vi "Test_pgJDP_built.vi"() -> ()   [LabVIEW 2020]
uses:
  <vilib>/Viviota/shared/ORM.lvlibp/TypeMap/TypeMap.lvclass
  <vilib>/Viviota/shared/ORM_pgsql_jdp.lvlibp/dbc/DBC.lvclass
  C:/Program Files/National Instruments/LabVIEW 2020/vi.lib/Viviota/shared/ORM.lvlibp/DbConnection/DbConnection.lvclass
  <vilib>/Viviota/shared/ORM_pgsql_jdp.lvlibp/PGJDPMapper/PGJDPMapper.lvclass
  C:/Program Files/National Instruments/LabVIEW 2020/vi.lib/Viviota/shared/ORM.lvlibp/SqlMapper/SqlMapper.lvclass
  <vilib>/Viviota/shared/ORM_lib.lvlibp/ObjectRow/ObjectLUT.lvclass
  <vilib>/numeric/Random Number (Range) I64.vi
  <vilib>/numeric/Random Number (Range) DBL.vi
  f3693442-7653-4e44-a421-498bef5f0c13.vi
  <vilib>/Analysis/baseanly.llb/Mean (DBL).vi
  <vilib>/numeric/sub_Random U32.vi
  <vilib>/JDP Science/JSONtext/Variant to JSON Text.vi
  <vilib>/Viviota/shared/ORM_lib.lvlibp/ObjectRow/Write LUT.vi
  <vilib>/Viviota/shared/ORM.lvlibp/DbConnection/Write SupportTX.vi
  <vilib>/Viviota/shared/ORM.lvlibp/SqlMapper/Write DbConnection.vi
  <vilib>/Viviota/shared/ORM.lvlibp/TypeMap/Write Table Name.vi
  <vilib>/Viviota/shared/ORM.lvlibp/TypeMap/Write Autokey.vi
  <vilib>/Viviota/shared/ORM_lib.lvlibp/ObjectRow/Read LUT.vi
  <vilib>/JDP Science/JSONtext/LVClass Serializer/JSONtext LVClass Serializer.lvclass
  <vilib>/Analysis/NI_AALBase.lvlib
panel:
  out "mean 3":dbl format="%0.6f"
  out "mean 2":dbl format="%0.6f"
  out "mean":dbl format="%0.6f"
  out "x-y":dbl[](array[numeric])
  out "Array 2":dbl[](array[numeric])
  out "Array":dbl[](array[numeric])
  out "LUT 2":variant[](array[variant])
  out "LUT":variant[](array[variant])
  out "id":i32[](array[numeric])
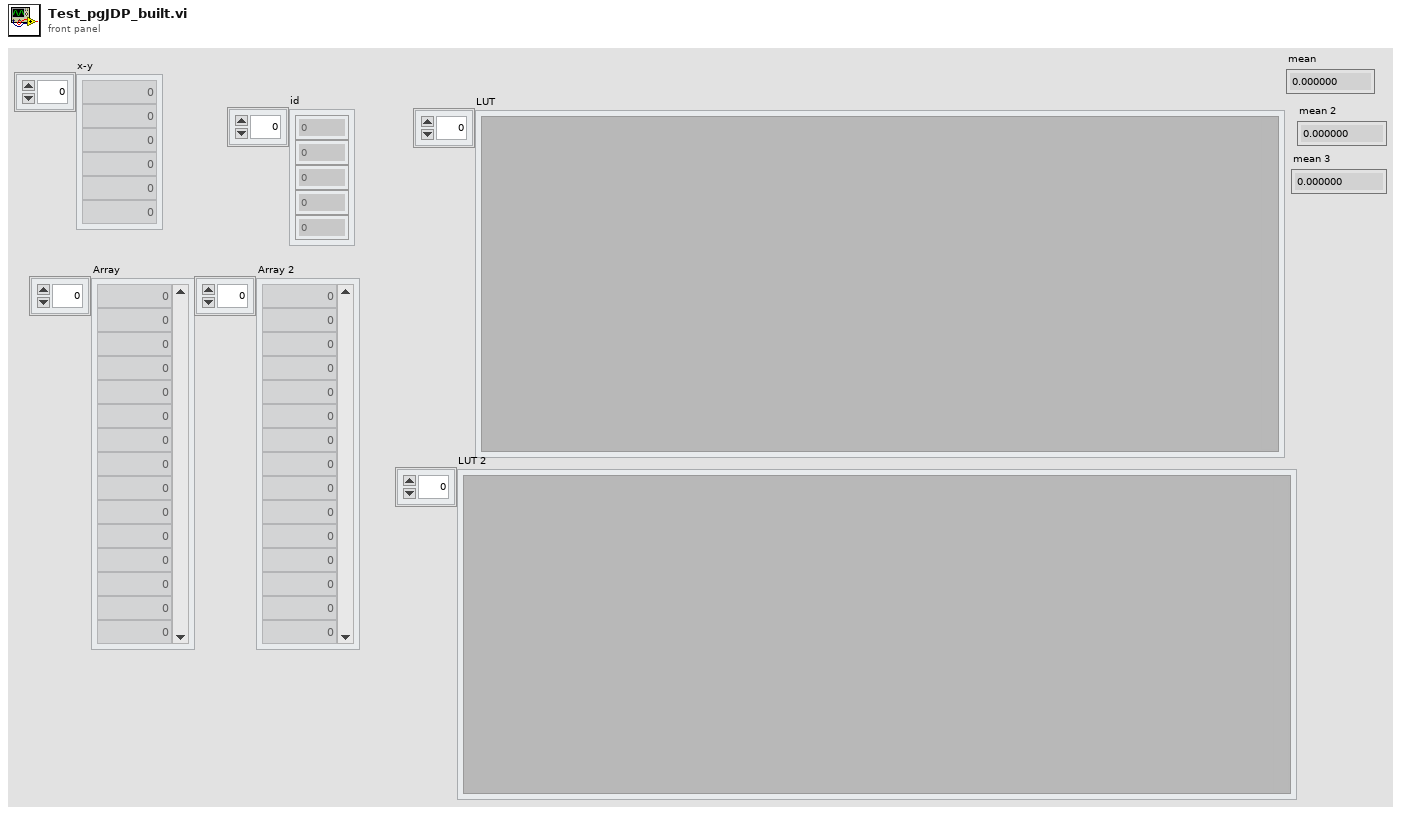
[diagram p1: front panel]
types:
  T1 = cluster{"Text":string, "Integer":i32, "dbl":dbl, "timestamp":timestamp}
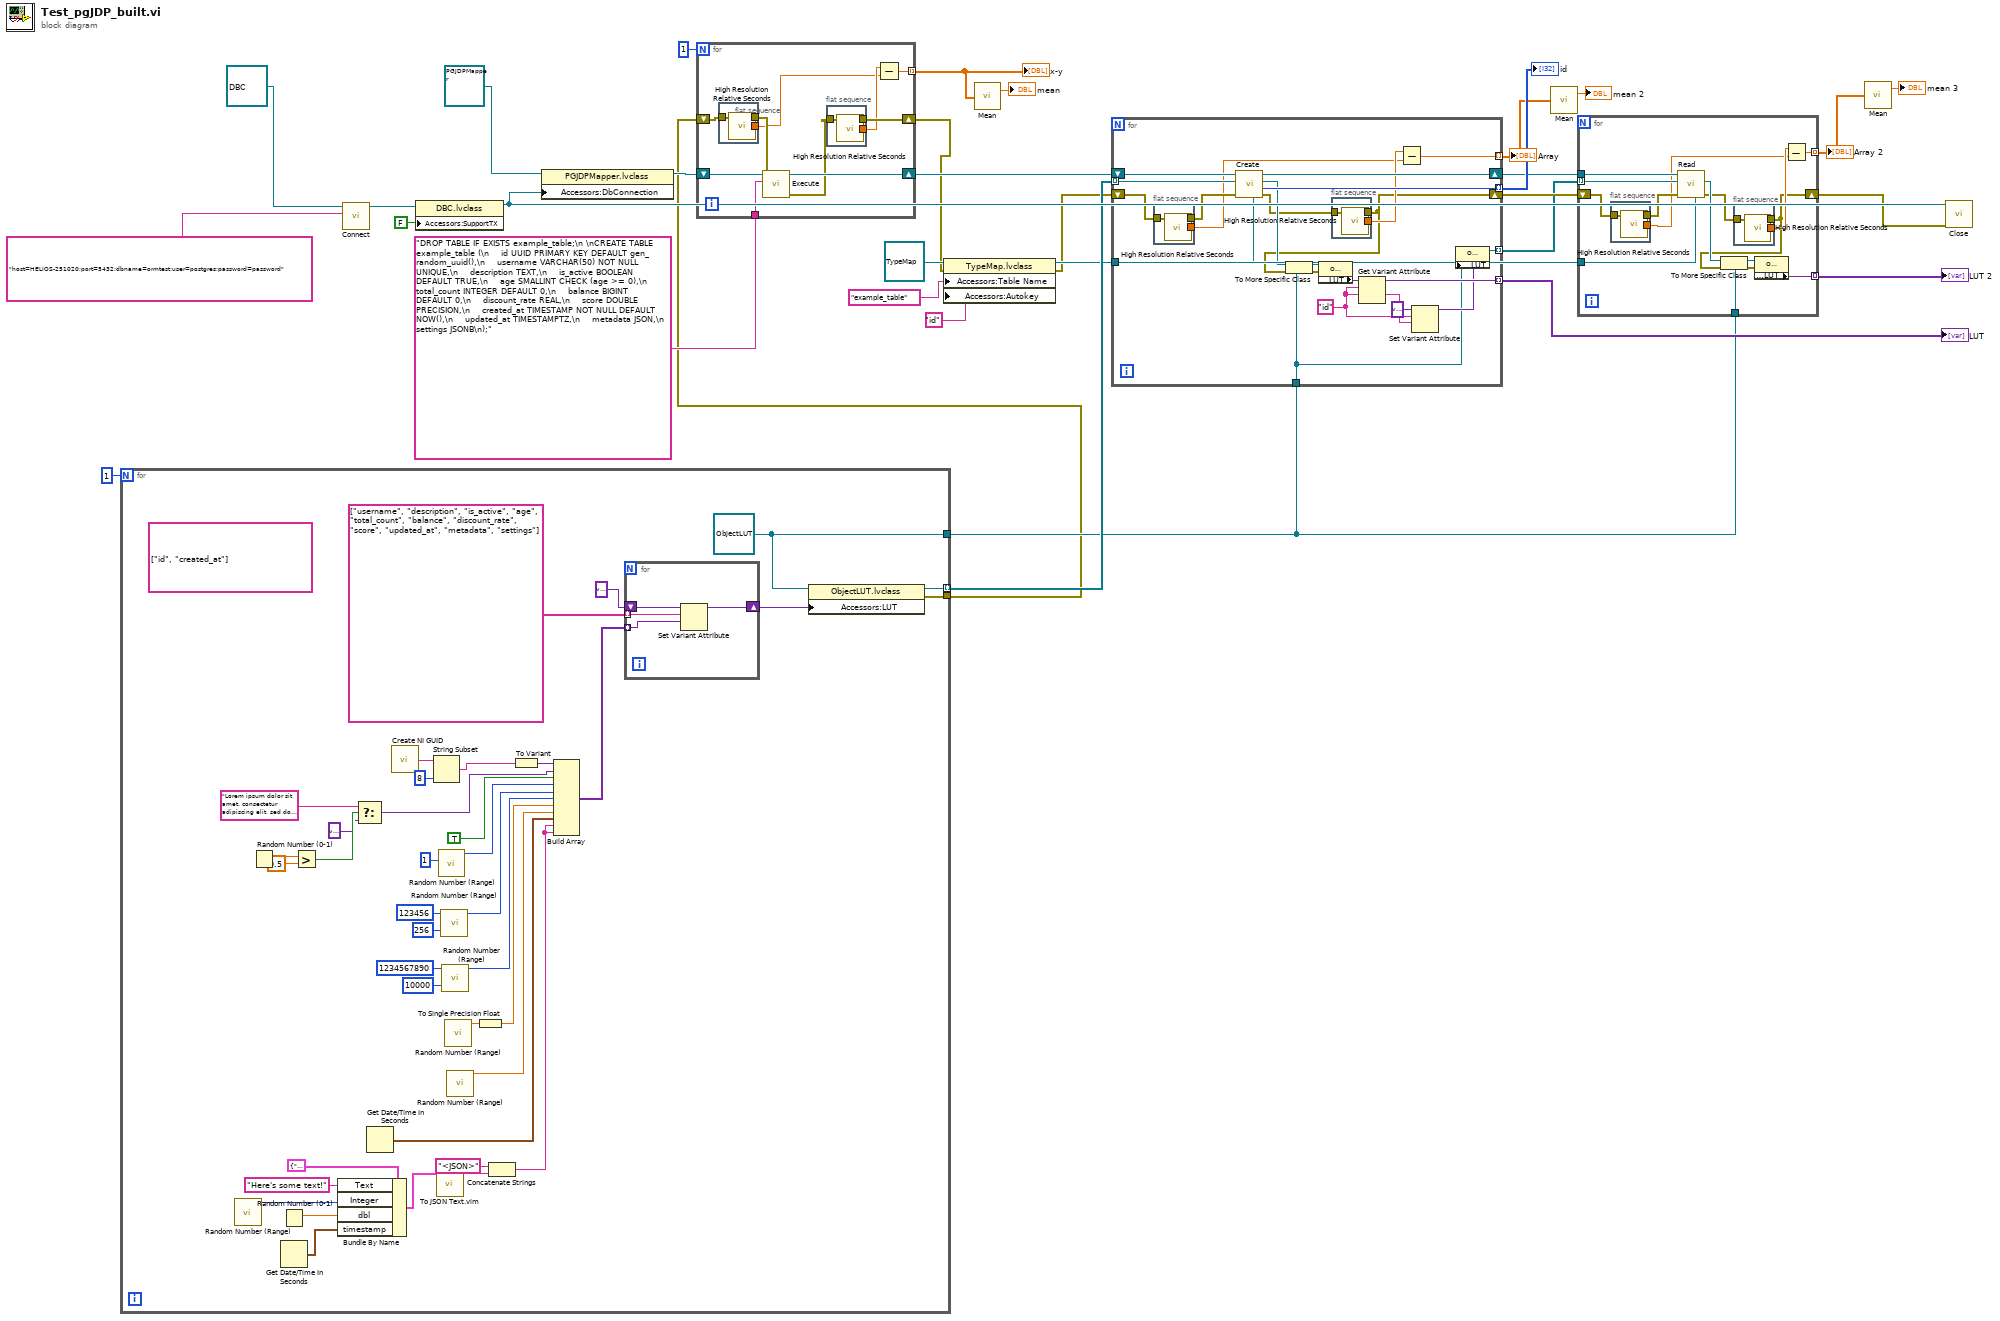
[diagram p0: block diagram]
diagram:
  n1 = for {
    N: 1 -> [_]
    tunnel: [w42] -> w27 mode=indexing
    tunnel: [w41] -> w17
    tunnel: [w36] -> w12
    w41 = refnum<class "ObjectLUT.lvclass"> refnum ("ORM_lib.lvlibp:ObjectLUT.lvclass")
    (unwired) string[] ["id", "created_at"]
    n2 = call-poly <vilib>:"Random Number (Range).vi"() -> ("number"=w49:i64)  [unwired: 11 in]
    n3 = Random Number (0-1)() -> (number: 0 to 1=w57:dbl)
    n4 = Random Number (0-1)() -> (number: 0 to 1=w50:dbl)
    n5 = Get Date/Time In Seconds() -> (seconds since 1Jan1904=w51:timestamp)
    n6 = Greater?(x=w57, y=0.5) -> (0:w55:bool)
    n7 = Bundle By Name(cluster=T1 {"Text"="This is a test", "Integer"=0, "dbl"=0.0, "timestamp"=timestamp(0 s since 1904-01-01)}, "Text"="Here's some text!", "Integer"=w49, "dbl"=w50, "timestamp"=w51) -> (w47:T1)
    n8 = Select(t="Lorem ipsum dolor sit amet, consectetur adipiscing elit, sed do eiusmod tempor incididunt ut labore et dolore magna aliqua", s=w55, f=variant) -> (s? t:f=w34:variant)
    n9 = Get Date/Time In Seconds() -> (seconds since 1Jan1904=w48:timestamp)
    n10 = call <vilib>:"Create NI GUID.vi"() -> ("NI GUID"=w72:string)
    n11 = String Subset(string=w72, length (rest)=8 ("length (rest)")) -> (substring=w67:string)  [unwired: 1 in]
    n12 = call "To JSON Text.vim"("Anything"=w47) -> ("<JSON>"=w40:string)  [unwired: 9 in, 1 out]
    n13 = call-poly <vilib>:"Random Number (Range).vi"("lower bound (-100)"=i64 1) -> ("number"=w64:i64)  [unwired: 10 in]
    n14 = call-poly <vilib>:"Random Number (Range).vi"("lower bound (-100)"=i64 256, "upper bound (100)"=i64 123456) -> ("number"=w63:i64)  [unwired: 9 in]
    n15 = call-poly <vilib>:"Random Number (Range).vi"("lower bound (-100)"=i64 10000, "upper bound (100)"=i64 1234567890) -> ("number"=w62:i64)  [unwired: 9 in]
    n16 = call-poly <vilib>:"Random Number (Range).vi"() -> ("number"=w60:dbl)  [unwired: 11 in]
    n17 = call-poly <vilib>:"Random Number (Range).vi"() -> ("number"=w58:dbl)  [unwired: 11 in]
    n18 = To Single Precision Float(number=w60) -> (single precision float=w59:sgl)
    n19 = Concatenate Strings("<JSON>" ("string"), w40) -> (w39:string)
    n20 = To Variant(anything=w67) -> (Variant=w66:variant)
    n21 = Build Array(w66, w34, TRUE, w64, w63, w62, w59, w58, w48, w39, w39) -> (w45:variant[])
    n22 = for {
      tunnel: string[] ["username", "description", "is_active", "age", "total_count", "balance", "discount_rate", "score", "updated_at", "metadata", "settings"] -> [w76] mode=indexing
      tunnel: w45 -> [w75] mode=indexing
      shift-right: [w74] -> w43
      shift-left: variant -> [w73]
      n23 = Set Variant Attribute(Variant=w73, name=w76, value=w75) -> (Variant out=w74:variant)  [unwired: 1 in, 2 out]
    }
    n24 = property class="ObjectLUT.lvclass"(reference=w41, "Accessors:LUT"=w43) -> (reference out=w42:refnum<class "ObjectLUT.lvclass">, error out=w36:errorcluster)  [unwired: 1 in]
  }
  n25 = call-dynamic "Connect.vi"("Connection String"="host=HELIOS-251020;port=5432;dbname=ormtest;user=postgres;password=password", "PostgresqlConnection in"=refnum<class "DBC.lvclass"> refnum ("ORM_pgsql_jdp.lvlibp:DBC.lvclass")) -> ("PostgresqlConnection out"=w32:refnum<class "DBC.lvclass">)  [unwired: 8 in, 1 out]
  n26 = property class="DBC.lvclass"(reference=w32, "Accessors:SupportTX"=FALSE ("SupportTX")) -> (reference out=w28:refnum<class "DBC.lvclass">)  [unwired: 1 in, 1 out]
  n27 = property class="PGJDPMapper.lvclass"(reference=refnum<class "PGJDPMapper.lvclass"> refnum ("ORM_pgsql_jdp.lvlibp:PGJDPMapper.lvclass"), "Accessors:DbConnection"=w28) -> (reference out=w30:refnum<class "PGJDPMapper.lvclass">)  [unwired: 1 in, 1 out]
  n28 = for {
    N: 1 -> [_]
    tunnel: "DROP TABLE IF EXISTS example_table;\n \nCREATE TABLE example_table (\n    id UUID PRIMARY KEY DEFAULT gen_random_uuid(),\n    username VARCHAR(50) NOT NULL UNIQUE,\n    description TEXT,\n    is_active BOOLEAN DEFAULT TRUE,\n    age SMALLINT CHECK (age >= 0),\n    total_count INTEGER DEFAULT 0,\n    balance BIGINT DEFAULT 0,\n    discount_rate REAL,\n    score DOUBLE PRECISION,\n    created_at TIMESTAMP NOT NULL DEFAULT NOW(),\n    updated_at TIMESTAMPTZ,\n    metadata JSON,\n    settings JSONB\n);" ("sql") -> [w85]
    tunnel: [w77] -> w9 mode=indexing
    shift-right: [w84] -> w19
    shift-left: w30 -> [w86]
    shift-right: [w80] -> w11
    shift-left: w12 -> [w83]
    n29 = flat-sequence {
      tunnel: [w90] -> w78
      tunnel: w83 -> [w89]
      tunnel: [w89] -> w82
      frame #0 {
        n30 = call <vilib>:"High Resolution Relative Seconds.vi"() -> ("relative seconds"=w90:dbl)
      }
    }
    n31 = call-dynamic "Execute.vi"("error in (no error)"=w82, "sql"=w85, "PGJDPMapper in"=w86) -> ("error out"=w81:errorcluster, "PGJDPMapper out"=w84:refnum<class "PGJDPMapper.lvclass">)  [unwired: 6 in, 1 out]
    n32 = flat-sequence {
      tunnel: [w88] -> w79
      tunnel: w81 -> [w87]
      tunnel: [w87] -> w80
      frame #0 {
        n33 = call <vilib>:"High Resolution Relative Seconds.vi"() -> ("relative seconds"=w88:dbl)
      }
    }
    n34 = Subtract(x=w79, y=w78) -> (x-y=w77:dbl)
  }
  "x-y" <- w9
  n35 = property class="TypeMap.lvclass"(reference=refnum<class "TypeMap.lvclass"> refnum ("TypeMap in"), error in=w11, "Accessors:Table Name"="example_table" ("Table Name"), "Accessors:Autokey"="id" ("Autokey")) -> (reference out=w18:refnum<class "TypeMap.lvclass">, error out=w3:errorcluster)
  n36 = call-poly <vilib>:"Mean.vi"("X"=w9) -> ("mean"=→"mean":dbl)  [unwired: 1 out]
  n37 = for {
    tunnel: w27 -> [w112] mode=indexing
    tunnel: w18 -> [w111]
    tunnel: [w110] -> w24 mode=indexing
    tunnel: w17 -> [w100]
    tunnel: [w105] -> w23 mode=indexing
    shift-right: [w91] -> w21
    shift-left: w3 -> [w98]
    tunnel: [w99] -> w20 mode=indexing
    shift-right: [w95] -> w13
    shift-left: w19 -> [w113]
    tunnel: [w92] -> w5 mode=indexing
    w103 = "id" ("name")
    n38 = flat-sequence {
      tunnel: [w117] -> w93
      tunnel: w98 -> [w116]
      tunnel: [w116] -> w97
      frame #0 {
        n39 = call <vilib>:"High Resolution Relative Seconds.vi"() -> ("relative seconds"=w117:dbl)
      }
    }
    n40 = call-dynamic "Create.vi"("TypeMap in"=w111, "error in (no error)"=w97, "object in"=w112, "SqlMapper in"=w113) -> ("error out"=w96:errorcluster, "id"=w110:i32, "object out"=w109:refnum<class>, "SqlMapper out"=w95:refnum<class "SqlMapper.lvclass">)  [unwired: 4 in]
    n41 = To More Specific Class(target class=w100, reference=w109, error in=w91) -> (specific class reference=w107:refnum<class "ObjectLUT.lvclass">, error out=w108:errorcluster)
    n42 = property class="ObjectLUT.lvclass"(reference=w107, error in=w108) -> ("Accessors:LUT"=w106:variant)  [unwired: 2 out]
    n43 = flat-sequence {
      tunnel: [w115] -> w94
      tunnel: w96 -> [w114]
      tunnel: [w114] -> w91
      frame #0 {
        n44 = call <vilib>:"High Resolution Relative Seconds.vi"() -> ("relative seconds"=w115:dbl)
      }
    }
    n45 = Get Variant Attribute(Variant=w106, name=w103, default value (empty Variant)=w103) -> (duplicate Variant=w105:variant, value=w102:string)  [unwired: 1 in, 2 out]
    n46 = Subtract(x=w94, y=w93) -> (x-y=w92:dbl)
    n47 = Set Variant Attribute(Variant=variant ("variant"), name=w103, value=w102) -> (Variant out=w101:variant)  [unwired: 1 in, 2 out]
    n48 = property class="ObjectLUT.lvclass"(reference=w100, "Accessors:LUT"=w101) -> (reference out=w99:refnum<class "ObjectLUT.lvclass">)  [unwired: 1 in, 1 out]
  }
  "id" <- w24
  "LUT" <- w23
  "Array" <- w5
  n49 = call-poly <vilib>:"Mean.vi"("X"=w5) -> ("mean"=→"mean 2":dbl)  [unwired: 1 out]
  n50 = for {
    tunnel: w20 -> [w132] mode=indexing
    tunnel: w13 -> [w131]
    tunnel: w18 -> [w130]
    tunnel: w17 -> [w126]
    tunnel: [w125] -> w16 mode=indexing
    shift-right: [w118] -> w15
    shift-left: w21 -> [w124]
    tunnel: [w119] -> w4 mode=indexing
    n51 = flat-sequence {
      tunnel: [w136] -> w120
      tunnel: w124 -> [w135]
      tunnel: [w135] -> w123
      frame #0 {
        n52 = call <vilib>:"High Resolution Relative Seconds.vi"() -> ("relative seconds"=w136:dbl)
      }
    }
    n53 = call-dynamic "Read.vi"("TypeMap in"=w130, "error in (no error)"=w123, "object in"=w132, "SqlMapper in"=w131) -> ("error out"=w122:errorcluster, "Value"=w127:refnum<class>)  [unwired: 4 in, 2 out]
    n54 = To More Specific Class(target class=w126, reference=w127, error in=w118) -> (specific class reference=w129:refnum<class "ObjectLUT.lvclass">, error out=w128:errorcluster)
    n55 = flat-sequence {
      tunnel: [w134] -> w121
      tunnel: w122 -> [w133]
      tunnel: [w133] -> w118
      frame #0 {
        n56 = call <vilib>:"High Resolution Relative Seconds.vi"() -> ("relative seconds"=w134:dbl)
      }
    }
    n57 = property class="ObjectLUT.lvclass"(reference=w129, error in=w128) -> ("Accessors:LUT"=w125:variant)  [unwired: 2 out]
    n58 = Subtract(x=w121, y=w120) -> (x-y=w119:dbl)
  }
  "LUT 2" <- w16
  "Array 2" <- w4
  n59 = call-poly <vilib>:"Mean.vi"("X"=w4) -> ("mean"=→"mean 3":dbl)  [unwired: 1 out]
  n60 = call-dynamic "Close.vi"("error in (no error)"=w15, "DBC in"=w28) -> ()  [unwired: 9 in, 1 out]
